vi "generate default line.vi"(8 "error in":errorcluster, 11 "objects in":T1) -> (0 "error out":errorcluster, 2 "Line":T2, 3 "objects out":T1)   [LabVIEW 2015, in "PID Module editor node.lvclass"]
doc: "Generates a new line with default settings."
uses:
  PID Module editor node.lvclass
  module/configuration/Line.ctl
  <vilib>/NI/Tag Bus Module Framework/channel/TBM channel.lvclass
  <vilib>/NI/DCAF/Tag Editor Core/Table API/Table Manager/object ref.ctl
  <vilib>/NI/DCAF/Tag Editor Core/Configuration Editor/Classes/Engine Parent/Engine Parent Editor Node.lvclass
  <vilib>/NI/DCAF/Tag Editor Core/Configuration Editor/Classes/Module editor node/module editor node.lvclass
  module/configuration/PID Module configuration.lvclass
  <vilib>/NI/Tag Bus/tag/tag descriptor.lvclass/tag descriptor.ctl
  <vilib>/NI/Tag Bus/tag/read tag name.vi
  <vilib>/NI/Configuration Framework/serializable configuration/NISE_CEF_serializable configuration.lvclass
  <vilib>/NI/Tag Bus/tag/tag descriptor.lvclass
  <vilib>/NI/DCAF/Tag Editor Core/Table API/Table Manager/Table Manager.lvclass
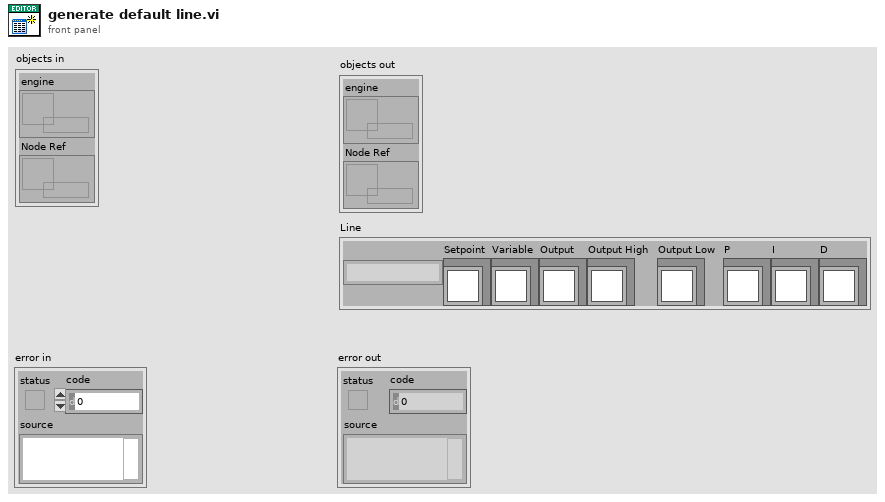
[diagram p1: front panel]
types:
  T1 = typedef "Table Manager.lvlib/Table Manager.lvclass/object ref.ctl" = cluster{"engine":refnum<data-value>, "Node Ref":refnum<data-value>}
  T2 = typedef "PID Module configuration.lvclass/Line.ctl" = cluster{"PID ID":string, "Setpoint":refnum<class "TBM channel.lvclass">, "Variable":refnum<class "TBM channel.lvclass">, "Output":refnum<class "TBM channel.lvclass">, "Output High":refnum<class "TBM channel.lvclass">, "Output Low":refnum<class "TBM channel.lvclass">, "P":refnum<class "TBM channel.lvclass">, "I":refnum<class "TBM channel.lvclass">, "D":refnum<class "TBM channel.lvclass">}
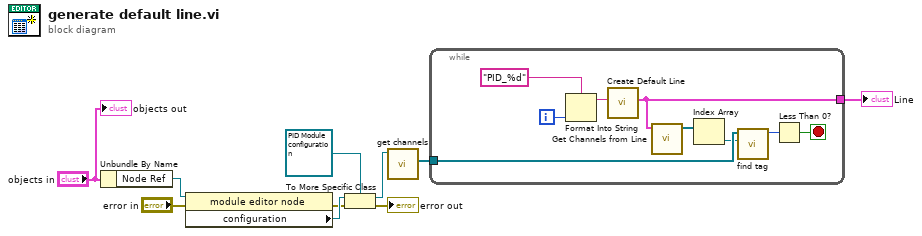
[diagram p0: block diagram]
diagram:
  n1 = Unbundle By Name("objects in") -> ("Node Ref"=w10:refnum<data-value>)
  n2 = property class="module editor node"(reference=w10, error in="error in") -> (error out=w4:errorcluster, "configuration"=w9:refnum<class "NISE_CEF_serializable configuration.lvclass">)  [unwired: 1 out]
  n3 = To More Specific Class(target class=refnum<class "PID Module configuration.lvclass"> refnum ("module configuration in"), reference=w9, error in=w4) -> (specific class reference=w8:refnum<class "PID Module configuration.lvclass">, error out=→"error out":errorcluster)
  n4 = call-dynamic "get channels.vi"("PID Module configuration in"=w8) -> ("channels"=w6:refnum<class "TBM channel.lvclass">[])  [unwired: 9 in, 1 out]
  n5 = while {
    tunnel: w6 -> [w14]
    tunnel: [w15] -> w1
    i -> [w19]
    stop <- w17 stop-if-true
    n6 = Format Into String(format string="PID_%d", w19) -> (resulting string=w16:string)  [unwired: 2 in, 1 out]
    n7 = call "Create Default Line.vi"("Line Name"=w16) -> ("Default Line"=w15:T2)  [unwired: 10 in]
    n8 = call "Get Channels from Line.vi"("Line"=w15) -> ("Channels"=w13:refnum<class "TBM channel.lvclass">[])  [unwired: 10 in]
    n9 = Index Array(array=w13) -> (element=w12:refnum<class "TBM channel.lvclass">)  [unwired: 1 in]
    n10 = call <vilib>:"find tag.vi"("tag"=w12, "tags in"=w14) -> ("index"=w11:i32)  [unwired: 9 in]
    n11 = Less Than 0?(x=w11) -> (x < 0?=w17:bool)
  }
  "Line" <- w1
  "objects out" <- "objects in"
